vi "Write Marker Value.vi"(8 "error in (no error)":errorcluster, 10 "Marker Value":T1 {"X-axis" format="%#_6p"}, 11 "Band Edge in":refnum<class "Band Edge.lvclass">) -> (0 "error out":errorcluster, 3 "Band Edge out":refnum<class "Band Edge.lvclass">)   [LabVIEW 2023, in "Spectrum Analyzer.lvlib" / "Band Edge.lvclass"]
uses:
  Band Edge.lvclass
  Band Edge.lvclass/Band Edge.ctl
  TYPE DEFINITION/TYPE Marker Value.ctl
  Spectrum Analyzer.lvlib
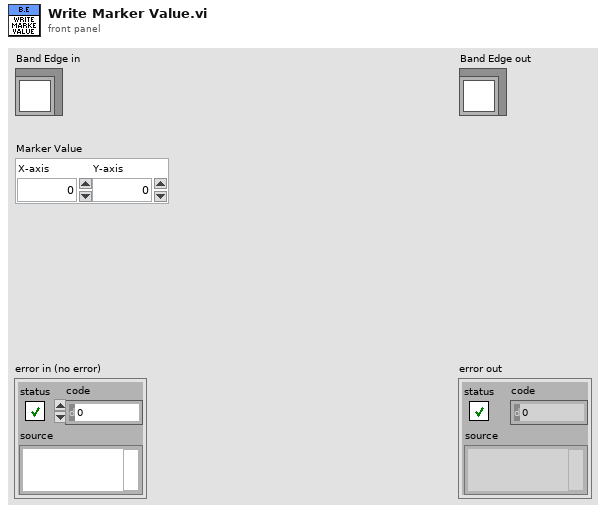
[diagram p1: front panel]
types:
  T1 = typedef "Spectrum Analyzer.lvlib/TYPE Marker Value.ctl" = cluster{"X-axis":dbl, "Y-axis":dbl}
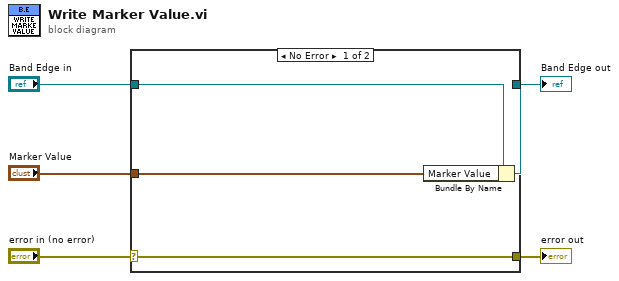
[diagram p0: block diagram]
diagram:
  n1 = case shown="No Error" "error in (no error)" {
    selector: "error in (no error)" -> [w9 w10]
    tunnel: [w9 w10] -> w4
    tunnel: [w7 w11] -> w2
    tunnel: "Band Edge in" -> [w8 w11]
    tunnel: "Marker Value" -> [w6 _]
    frame No Error {
      n2 = Bundle By Name(cluster=w8, "Marker Value"=w6) -> (w7:refnum<class "Band Edge.lvclass">)
    }
    frame Error {
    }
  }
  "error out" <- w4
  "Band Edge out" <- w2
